vi "VIH ProjFile - HHP Generation - Write.vi"(5 "Build Root Dir":path, 7 "Project Folder":path, 8 "error in":errorcluster, 9 "HHP_Generation":T1={"HHP_Template"=enum."default", "HHP_Template_CustomPath"=path "", "HHP_Target"=enum."default", "HHP_Target_CustomPath"=path "", "HHP_CreateTOC"=TRUE, "HHP_CreateIDX"=TRUE, "HHP_DefaultTopic"=enum."auto", "HHP_DefaultTopic_CustomPath"=path "", "CHM_Filename"=path "", "HHP_AutoBuild"=FALSE, "CHM_AutoBuild"=FALSE}, 11 "XML Parent Item":refnum<k20>) -> (0 "error out":errorcluster, 3 "dup XML Parent Item":refnum<k20>)   [LabVIEW 2014]
doc: "::: VI Helpeks :::\nCopyright (c) 2000-2026 Konstantin Shifershteyn. All rights reserved."
uses:
  _VIH CHM Project.llb/VIH - CHM Project - HHP Generation Params Cluster.ctl
  <vilib>/xml/Close Reference(Node).vi
  <resource>/objmgr/DOMUserDefRef.rc
  <vilib>/xml/NI_XML.lvlib
panel:
  in  "HHP_Generation (data)":T1={"HHP_Template"=enum."default", "HHP_Template_CustomPath"=path "", "HHP_Target"=enum."default", "HHP_Target_CustomPath"=path "", "HHP_CreateTOC"=TRUE, "HHP_CreateIDX"=TRUE, "HHP_DefaultTopic"=enum."auto", "HHP_DefaultTopic_CustomPath"=path "", "CHM_Filename"=path "", "HHP_AutoBuild"=FALSE, "CHM_AutoBuild"=FALSE}
  # "VI Helpeks\nCopyright (c) 2012-2026 Konstantin Shifershteyn"
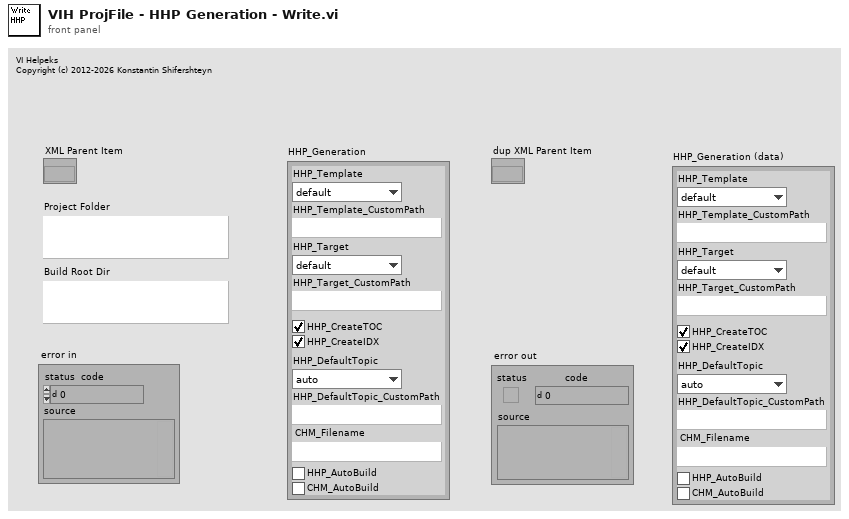
[diagram p1: front panel]
types:
  T1 = typedef "VIH - CHM Project - HHP Generation Params Cluster.ctl" = cluster{"HHP_Template":enum16{"default", "custom"}, "HHP_Template_CustomPath":path, "HHP_Target":enum16{"default", "custom"}, "HHP_Target_CustomPath":path, "HHP_CreateTOC":bool, "HHP_CreateIDX":bool, "HHP_DefaultTopic":enum16{"auto", "custom"}, "HHP_DefaultTopic_CustomPath":path, "CHM_Filename":path, "HHP_AutoBuild":bool, "CHM_AutoBuild":bool}
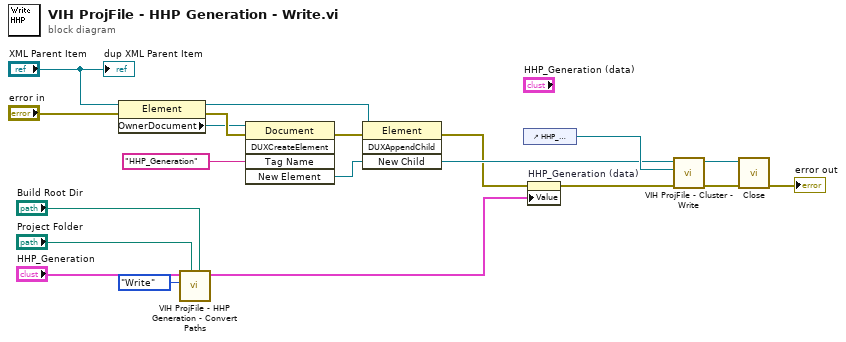
[diagram p0: block diagram]
diagram:
  n1 = property class="Element"(reference="XML Parent Item", error in="error in") -> (reference out=w10:refnum<k20>, error out=w12:errorcluster, "OwnerDocument"=w9:refnum<k20>)
  n2 = call "VIH ProjFile - HHP Generation - Convert Paths.vi"("Build Root Dir"="Build Root Dir", "Project Dir"="Project Folder", "Operation"=enum16{"Read", "Write"}."Write", "HHP_Generation"="HHP_Generation") -> ("HHP_Generation out"=w8:T1)  [unwired: 7 in]
  n3 = invoke class="Document" method="DUXCreateElement"(reference=w9, error in=w12, "Tag Name"="HHP_Generation") -> (error out=w14:errorcluster, "New Element"=w18:refnum<k20>)  [unwired: 2 in, 3 out]
  n4 = invoke class="Element" method="DUXAppendChild"(reference=w10, error in=w14, "New Child"=w18) -> (error out=w16:errorcluster)  [unwired: 1 in, 3 out]
  n5 = control-ref of="HHP_Generation (data)"() -> (w19:refnum<vi>)
  n6 = property on="HHP_Generation (data)" class="Clust (strict)"(error in=w16, "Value"=w8) -> (error out=w17:errorcluster)  [unwired: 1 in, 1 out]
  n7 = call "VIH ProjFile - Cluster - Write.vi"("error in"=w17, "Ctl Refnum"=w19, "XML Parent Item"=w18) -> ("error out"=w3:errorcluster, "dup XML Parent Item"=w4:refnum<k20>)  [unwired: 7 in]
  n8 = call-poly <vilib>:"Close.vi"("error in (no error)"=w3, "node"=w4) -> ("error out"=→"error out":errorcluster)  [unwired: 7 in]
  "dup XML Parent Item" <- "XML Parent Item"
